vi "Controller Algorithm.vi"(6 "EventLog":refnum<class "abs_EventLog.lvclass">, 8 "Heater Output":refnum<class "Abs_Boolean.lvclass">, 9 "Lower Limit":refnum<class "Abs_Double Float.lvclass">, 10 "Upper Limit":refnum<class "Abs_Double Float.lvclass">, 11 "Reading":refnum<class "Abs_Double Float.lvclass">) -> (3 "Node Out":refnum<class "bt_Node.lvclass">)   [LabVIEW 2021]
uses:
  Support/Nodes/abs_Node/bt_Node.lvclass
  <vilib>/TSA/Abstract Data Classes/Abs_Types/Double Float/Abs_Double Float.lvclass
  C:/Program Files (x86)/National Instruments/LabVIEW 2021/vi.lib/TSA/Abstract Data Classes/Abs_Types/Numeric/Abs_Numeric.lvclass
  <vilib>/TSA/Abstract Data Classes/Abs_Types/Boolean/Abs_Boolean.lvclass
  C:/Program Files (x86)/National Instruments/LabVIEW 2021/vi.lib/TSA/Abstract Data Classes/Abs_Types/Value/Abs_Value.lvclass
  C:/Program Files (x86)/National Instruments/LabVIEW 2021/vi.lib/TSA/Abstract Data Classes/Abs_Types/Type/Abs_Type.lvclass
  <vilib>/TSA/Event Log/abs_EventLog/abs_EventLog.lvclass
  Support/Nodes/Leaves/abs_Type Leaf/abs_Type Leaf.lvclass/abs_Type Leaf.ctl
  Support/Nodes/Leaves/abs_Type Leaf/Properties/Write Value Class.vi
  Support/Nodes/Leaves/Test Boolean/Test Abs_Boolean.lvclass
  C:/Users/timst/Documents/Repositories/LV_Behaviour_Tree/Source/Support/Nodes/abs_Node/bt_Node.lvclass
  C:/Users/timst/Documents/Repositories/LV_Behaviour_Tree/Source/Support/Nodes/Leaves/abs_Type Leaf/abs_Type Leaf.lvclass
  Support/Nodes/Leaves/Log/bt_Log.lvclass
  <vilib>/TSA/Abstract Data Classes/Functions/Compare/Support/Greater/DBL/Method.vi
  <vilib>/TSA/Abstract Data Classes/Functions/Compare/Support/Less/DBL/Method.vi
  <vilib>/TSA/Abstract Data Classes/Constants/Support/Bool/Bool.vi
  <vilib>/TSA/Abstract Data Classes/Constants/Support/Str/Str.vi
  BT.lvlib
  C:/Program Files (x86)/National Instruments/LabVIEW 2021/vi.lib/TSA/Abstract Data Classes/Abs_Types/Floating Point/Abs_Floating Point.lvclass
  C:/Program Files (x86)/National Instruments/LabVIEW 2021/vi.lib/TSA/Abstract Data Classes/Abs_Types/Double Float/Abs_Double Float.lvclass
  <vilib>/TSA/Abstract Data Classes/Constants/Support/Bool/Const_Bool.lvclass
  <vilib>/TSA/Abstract Data Classes/Functions/Compare/Support/Greater/DBL/Greater_DBL.lvclass
  <vilib>/TSA/Abstract Data Classes/Functions/Compare/Support/Less/DBL/Less_DBL.lvclass
  <vilib>/TSA/Abstract Data Classes/Constants/Support/Str/Const_Str.lvclass
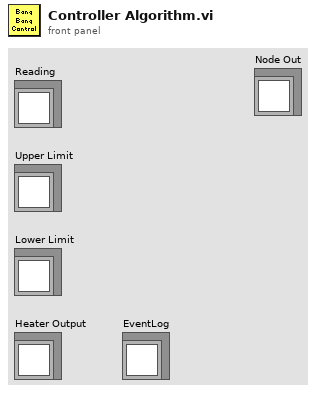
[diagram p1: front panel]
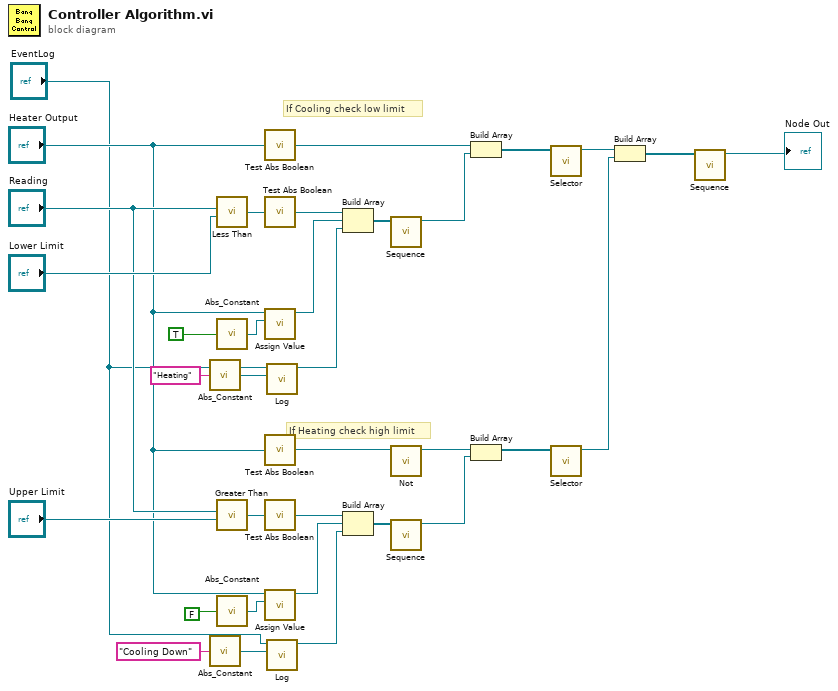
[diagram p0: block diagram]
diagram:
  # "If Heating check high limit"
  # "If Cooling check low limit"
  n1 = call-poly <vilib>:"Abs_Constant.vi"("String"="Heating") -> ("Abs_String.lvclass"=w6:refnum<class "Abs_String.lvclass">)  [unwired: 4 in]
  n2 = call-poly <vilib>:"Abs_Constant.vi"("String"="Cooling Down") -> ("Abs_String.lvclass"=w3:refnum<class "Abs_String.lvclass">)  [unwired: 4 in]
  n3 = call-poly <vilib>:"Less Than.vi"("Value B"="Lower Limit", "Value A"="Reading") -> ("Result"=w20:refnum<class "Abs_Boolean.lvclass">)  [unwired: 4 in]
  n4 = call-poly <vilib>:"Abs_Constant.vi"("Boolean"=TRUE ("Boolean Value")) -> ("Abs_Boolean.lvclass"=w12:refnum<class "Abs_Boolean.lvclass">)  [unwired: 4 in]
  n5 = call-poly <vilib>:"Greater Than.vi"("Value B"="Upper Limit", "Value A"="Reading") -> ("Result"=w16:refnum<class "Abs_Boolean.lvclass">)  [unwired: 4 in]
  n6 = call-poly <vilib>:"Abs_Constant.vi"("Boolean"=FALSE ("Boolean Value")) -> ("Abs_Boolean.lvclass"=w9:refnum<class "Abs_Boolean.lvclass">)  [unwired: 4 in]
  n7 = call "Test Abs Boolean.vi"("Abs_Boolean.lvclass"="Heater Output") -> ("abs_Node"=w24:refnum<class "bt_Node.lvclass">)  [unwired: 4 in]
  n8 = call "Test Abs Boolean.vi"("Abs_Boolean.lvclass"=w20) -> ("abs_Node"=w21:refnum<class "bt_Node.lvclass">)  [unwired: 4 in]
  n9 = call "Assign Value.vi"("Assigned Value"=w12, "Value"="Heater Output") -> ("Node Out"=w11:refnum<class "bt_Node.lvclass">)  [unwired: 9 in]
  n10 = call "Test Abs Boolean.vi"("Abs_Boolean.lvclass"="Heater Output") -> ("abs_Node"=w23:refnum<class "bt_Node.lvclass">)  [unwired: 4 in]
  n11 = call "Test Abs Boolean.vi"("Abs_Boolean.lvclass"=w16) -> ("abs_Node"=w15:refnum<class "bt_Node.lvclass">)  [unwired: 4 in]
  n12 = call "Assign Value.vi"("Assigned Value"=w9, "Value"="Heater Output") -> ("Node Out"=w13:refnum<class "bt_Node.lvclass">)  [unwired: 9 in]
  n13 = call "Log.vi"("Message"=w6, "EventLog"="EventLog") -> ("node out"=w7:refnum<class "bt_Log.lvclass">)  [unwired: 9 in]
  n14 = call "Log.vi"("Message"=w3, "EventLog"="EventLog") -> ("node out"=w2:refnum<class "bt_Log.lvclass">)  [unwired: 9 in]
  n15 = Build Array(w21, w11, w7) -> (w33:refnum<class "bt_Node.lvclass">[])
  n16 = Build Array(w15, w13, w2) -> (w28:refnum<class "bt_Node.lvclass">[])
  n17 = call "Sequence.vi"("Nodes"=w33) -> ("Node"=w32:refnum<class "bt_Node.lvclass">)  [unwired: 10 in]
  n18 = call "Not.vi"("Node In"=w23) -> ("Node"=w22:refnum<class "bt_Node.lvclass">)  [unwired: 10 in]
  n19 = call "Sequence.vi"("Nodes"=w28) -> ("Node"=w29:refnum<class "bt_Node.lvclass">)  [unwired: 10 in]
  n20 = Build Array(w24, w32) -> (w34:refnum<class "bt_Node.lvclass">[])
  n21 = Build Array(w22, w29) -> (w26:refnum<class "bt_Node.lvclass">[])
  n22 = call "Selector.vi"("Nodes"=w34) -> ("Node"=w31:refnum<class "bt_Node.lvclass">)  [unwired: 10 in]
  n23 = call "Selector.vi"("Nodes"=w26) -> ("Node"=w25:refnum<class "bt_Node.lvclass">)  [unwired: 10 in]
  n24 = Build Array(w31, w25) -> (w30:refnum<class "bt_Node.lvclass">[])
  n25 = call "Sequence.vi"("Nodes"=w30) -> ("Node"=→"Node Out":refnum<class "bt_Node.lvclass">)  [unwired: 10 in]
